vi "Lost_Error.vi"(8 "cause":errorcluster, 11 "operation":string) -> (0 "error out":errorcluster)   [LabVIEW 2021, in "CANsub_API.lvlib"]
doc: "Makes error 5203 (connection lost) and keeps the original error code and source in the message. Loop-safe: no allocation, bounded time."
uses:
  CANsub_API.lvlib
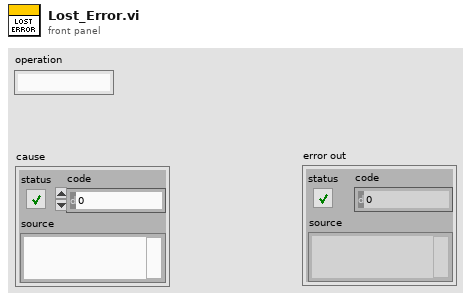
[diagram p1: front panel]
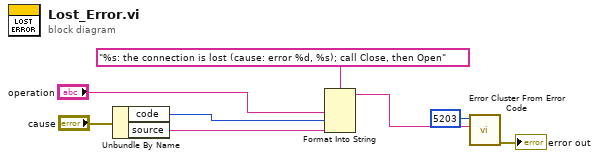
[diagram p0: block diagram]
diagram:
  n1 = Unbundle By Name("cause") -> ("code"=w5:i32, "source"=w4:string)
  n2 = Format Into String(format string="%s: the connection is lost (cause: error %d, %s); call Close, then Open", "operation", w5, w4) -> (resulting string=w2:string)  [unwired: 2 in, 1 out]
  n3 = call <vilib>:"Error Cluster From Error Code.vi"("error message (\"\")"=w2, "error code (0)"=5203) -> ("error out"=→"error out":errorcluster)  [unwired: 7 in]
